vi "OrderSpectrumToFlexLogger.vi"(7 "Spectrum Display Settings":T1={"channels"=1, "plot points per block"=641, "plot in dB? (F)"=FALSE, "window ENBW (bins)"=1.5}, 8 "error in (no error)":errorcluster, 9 "reset? (F)":bool, 10 "Timing Reference":waveform(dbl), 11 "order power spectra":T2(array[cluster])) -> (0 "error out":errorcluster, 1 "Log Values":dbl[](array[numeric]), 2 "Log Waveforms":waveform(dbl)[](array[waveform]), 3 "Plot Waveforms":waveform(dbl)[](array[waveform]), 4 "Plot Values":dbl[][](array[numeric]))   [LabVIEW 2026]
doc: "Turns an order power spectrum (OAT Order Power Spectrum output, linear power EU^2 rms, dB on? = FALSE) into FlexLogger channels for the plug-in Process.vi.\norder power spectra = 1D array of {order 0, delta order, magnitude}, one element per channel (Build Array the single-channel output). An empty magnitude (no new spectrum this block) keeps the last spectrum, so every channel is written every block.\nTiming Reference = any input waveform of this block (t0 and block length).\nPlot Waveforms (to Write 1D Wfm, Auto Calculate T0 = TRUE): Order Axis, then one Order Spectrum per channel. Each is a burst of 'plot points per block' points per block, dt = block length / plot points. On a FlexLogger XY Graph map Order Axis to X and Order Spectrum to Y. Points past the last bin repeat the last bin.\nLog Waveforms: 1-point waveforms, dt = block length: Spectrum Valid (0/1), Spectrum Count (spectra since reset), Order Resolution, Max Order, then per channel Overall Level (EU rms over the whole order range, divided by window ENBW), Peak Order, Peak Amplitude (EU rms of the highest bin).\nLog Values and Plot Values carry the same numbers as plain arrays (for tests).\nreset? TRUE on the first Process call after Configure Session clears the held spectrum and the count."
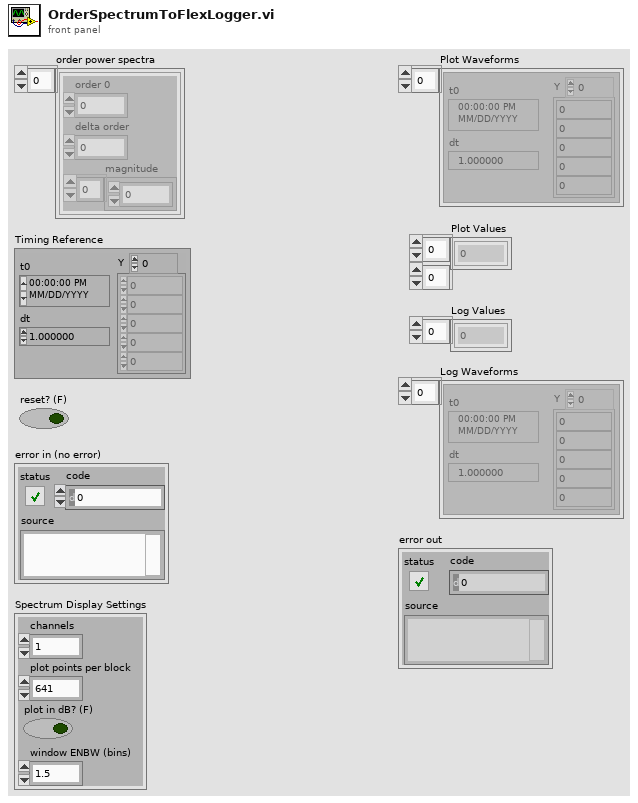
[diagram p1: front panel]
types:
  T1 = cluster{"channels":i32, "plot points per block":i32, "plot in dB? (F)":bool, "window ENBW (bins)":dbl}
  T2 = cluster{"order 0":dbl, "delta order":dbl, "magnitude":dbl[]}[]
  T3 = cluster{"order 0":dbl, "delta order":dbl, "magnitude":dbl[]}
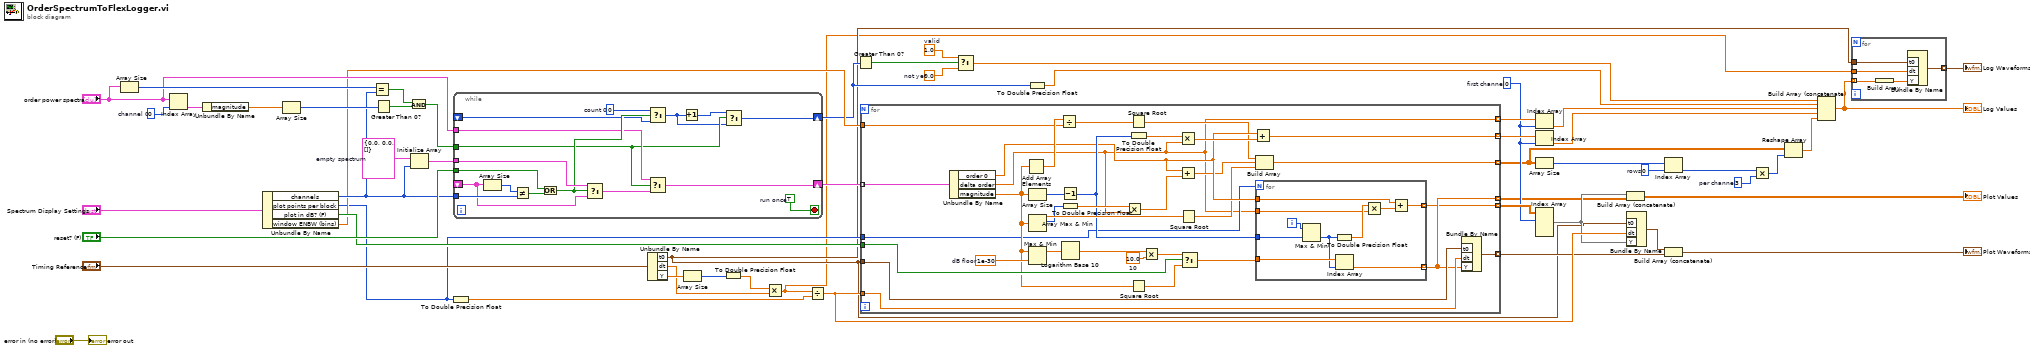
[diagram p0: block diagram]
diagram:
  w13 = 3  # per channel
  w15 = 0  # rows
  w18 = 0.0  # not yet
  w20 = 1.0  # valid
  w28 = 0  # first channel
  w47 = T3 {"order 0"=0.0, "delta order"=0.0, "magnitude"=[]}  # empty spectrum
  w53 = 0  # channel 0
  n1 = Array Size(array="order power spectra") -> (size(s)=w54:i32)
  n2 = Index Array(array="order power spectra", index=w53) -> (element=w52:T3)
  n3 = Unbundle By Name(w52) -> ("magnitude"=w51:dbl[])
  n4 = Unbundle By Name("Spectrum Display Settings") -> ("channels"=w42:i32, "plot points per block"=w32:i32, "plot in dB? (F)"=w34:bool, "window ENBW (bins)"=w33:dbl)
  n5 = Array Size(array=w51) -> (size(s)=w50:i32)
  n6 = Equal?(x=w54, y=w42) -> (x = y?=w49:bool)
  n7 = Greater Than 0?(x=w50) -> (x > 0?=w48:bool)
  n8 = And(x=w49, y=w48) -> (x .and. y?=w45:bool)
  n9 = Initialize Array(w47, w42) -> (w43:T2)
  n10 = To Double Precision Float(number=w32) -> (double precision float=w36:dbl)
  n11 = while {
    tunnel: "order power spectra" -> [w63]
    tunnel: w45 -> [w59]
    tunnel: "reset? (F)" -> [w70]
    tunnel: w43 -> [w68]
    tunnel: w42 -> [w71]
    shift-right: [w61] -> w35
    shift-left: _ -> [w67]
    shift-right: [w57] -> w17
    shift-left: _ -> [w64]
    stop <- w56 stop-if-true
    w56 = TRUE  # run once
    w66 = 0  # count 0
    n12 = Array Size(array=w67) -> (size(s)=w72:i32)
    n13 = Not Equal?(x=w72, y=w71) -> (x != y?=w69:bool)
    n14 = Or(x=w70, y=w69) -> (x .or. y?=w65:bool)
    n15 = Select(t=w68, s=w65, f=w67) -> (s? t:f=w62:T2)
    n16 = Select(t=w63, s=w59, f=w62) -> (s? t:f=w61:T2)
    n17 = Select(t=w66, s=w65, f=w64) -> (s? t:f=w58:i32)
    n18 = Increment(x=w58) -> (x+1=w60:i32)
    n19 = Select(t=w60, s=w59, f=w58) -> (s? t:f=w57:i32)
  }
  n20 = Unbundle By Name("Timing Reference") -> ("t0"=w4:timestamp, "dt"=w37:dbl, "Y"=w40:dbl[])
  n21 = Array Size(array=w40) -> (size(s)=w39:i32)
  n22 = To Double Precision Float(number=w39) -> (double precision float=w38:dbl)
  n23 = Multiply(x=w38, y=w37) -> (x*y=w3:dbl)
  n24 = Divide(x=w3, y=w36) -> (x/y=w27:dbl)
  n25 = Greater Than 0?(x=w17) -> (x > 0?=w19:bool)
  n26 = for {
    tunnel: w35 -> [w106] mode=indexing
    tunnel: w34 -> [w100]
    tunnel: w33 -> [w97]
    tunnel: w32 -> [w84]
    tunnel: w4 -> [w83]
    tunnel: w27 -> [w82]
    tunnel: [w78] -> w25 mode=indexing
    tunnel: [w77] -> w22 mode=indexing
    tunnel: [w76] -> w31 mode=indexing
    tunnel: [w75] -> w12 mode=indexing
    tunnel: [w74] -> w30 mode=indexing
    tunnel: [w73] -> w29 mode=indexing
    w102 = 10.0  # 10
    w105 = 1e-30  # dB floor
    n27 = Unbundle By Name(w106) -> ("order 0"=w85:dbl, "delta order"=w74:dbl, "magnitude"=w95:dbl[])
    n28 = Add Array Elements(numeric array=w95) -> (sum=w98:dbl)
    n29 = Array Size(array=w95) -> (size(s)=w90:i32)
    n30 = Array Max & Min(array=w95) -> (max value=w94:dbl, max index (indices)=w93:i32)  [unwired: 2 out]
    n31 = Max & Min(x=w95, y=w105) -> (max(x,y)=w104:dbl[])  [unwired: 1 out]
    n32 = Divide(x=w98, y=w97) -> (x/y=w96:dbl)
    n33 = Decrement(x=w90) -> (x-1=w86:i32)
    n34 = To Double Precision Float(number=w93) -> (double precision float=w92:dbl)
    n35 = Logarithm Base 10(1:w104) -> (0:w103:dbl[])
    n36 = Multiply(x=w92, y=w74) -> (x*y=w91:dbl)
    n37 = Square Root(x=w96) -> (sqrt(x)=w81:dbl)
    n38 = To Double Precision Float(number=w86) -> (double precision float=w89:dbl)
    n39 = Square Root(x=w95) -> (sqrt(x)=w99:dbl[])
    n40 = Multiply(x=w103, y=w102) -> (x*y=w101:dbl[])
    n41 = Multiply(x=w89, y=w74) -> (x*y=w88:dbl)
    n42 = Add(x=w85, y=w91) -> (x+y=w80:dbl)
    n43 = Square Root(x=w94) -> (sqrt(x)=w79:dbl)
    n44 = Select(t=w101, s=w100, f=w99) -> (s? t:f=w87:dbl[])
    n45 = Add(x=w85, y=w88) -> (x+y=w73:dbl)
    n46 = Build Array(w81, w80, w79) -> (w75:dbl[])
    n47 = for {
      N: w84 -> [_]
      tunnel: w87 -> [w115]
      tunnel: w86 -> [w116]
      tunnel: w85 -> [w111]
      tunnel: w74 -> [w112]
      tunnel: [w109] -> w77 mode=indexing
      tunnel: [w108] -> w76 mode=indexing
      i -> [w107]
      n48 = Max & Min(x=w107, y=w116) -> (min(x,y)=w114:i32)  [unwired: 1 out]
      n49 = To Double Precision Float(number=w114) -> (double precision float=w113:dbl)
      n50 = Index Array(array=w115, index=w114) -> (element=w109:dbl)
      n51 = Multiply(x=w113, y=w112) -> (x*y=w110:dbl)
      n52 = Add(x=w111, y=w110) -> (x+y=w108:dbl)
    }
    n53 = Bundle By Name("t0"=w83, "dt"=w82, "Y"=w77) -> (w78:waveform(dbl))  [unwired: 1 in]
  }
  n54 = Select(t=w20, s=w19, f=w18) -> (s? t:f=w10:dbl)
  n55 = To Double Precision Float(number=w17) -> (double precision float=w9:dbl)
  n56 = Index Array(array=w30, index=w28) -> (element=w8:dbl)
  n57 = Index Array(array=w29, index=w28) -> (element=w7:dbl)
  n58 = Array Size(array=w12) -> (size(s)=w16:i32[])
  n59 = Index Array(array=w31, index (row) #1=w28) -> (element #1=w23:dbl[])  [unwired: 3 in, 1 out]
  n60 = Bundle By Name("t0"=w4, "dt"=w27, "Y"=w23) -> (w26:waveform(dbl))  [unwired: 1 in]
  n61 = Build Array (concatenate)(w23, w22) -> (→"Plot Values":dbl[][])
  n62 = Index Array(array=w16, index=w15) -> (element=w14:i32)
  n63 = Build Array (concatenate)(w26, w25) -> (→"Plot Waveforms":waveform(dbl)[])
  n64 = Multiply(x=w14, y=w13) -> (x*y=w11:i32)
  n65 = Reshape Array(w12, w11) -> (w6:dbl[])
  n66 = Build Array (concatenate)(w10, w9, w8, w7, w6) -> (w5:dbl[])
  "Log Values" <- w5
  n67 = for {
    tunnel: w5 -> [w121] mode=indexing
    tunnel: w4 -> [w120]
    tunnel: w3 -> [w119]
    tunnel: [w117] -> w2 mode=indexing
    n68 = Build Array(w121) -> (w118:dbl[])
    n69 = Bundle By Name("t0"=w120, "dt"=w119, "Y"=w118) -> (w117:waveform(dbl))  [unwired: 1 in]
  }
  "Log Waveforms" <- w2
  "error out" <- "error in (no error)"
